vi "VIH HelpGen - HTML - Path to String.vi"(11 "Path":path) -> (3 "String":string)   [LabVIEW 2014]
doc: "::: VI Helpeks :::\nCopyright (c) 2000-2026 Konstantin Shifershteyn. All rights reserved."
panel:
  # "VI Helpeks\nCopyright (c) 2012-2026 Konstantin Shifershteyn"
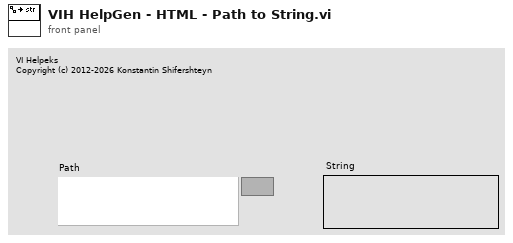
[diagram p1: front panel]
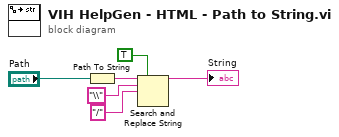
[diagram p0: block diagram]
diagram:
  n1 = Path To String(path="Path") -> (string=w6:string)
  n2 = Search and Replace String(replace all?=TRUE, input string=w6, search string="\\", replace string="/") -> (result string=→"String":string)  [unwired: 4 in, 3 out]
